vi "VIH Platform - LabVIEW - Read Show_Optional_Terminals status in Context Help.vi"(8 "error in":errorcluster) -> (0 "error out":errorcluster, 3 "simpleDiagramHelp (Hide Optional Terminals)":bool)   [LabVIEW 2014]
doc: "::: VI Helpeks :::\nCopyright (c) 2000-2026 Konstantin Shifershteyn. All rights reserved."
panel:
  # "VI Helpeks\nCopyright (c) 2012-2026 Konstantin Shifershteyn"
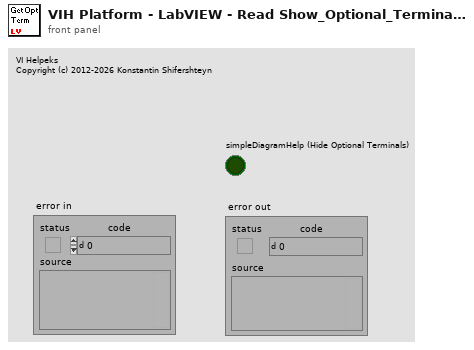
[diagram p1: front panel]
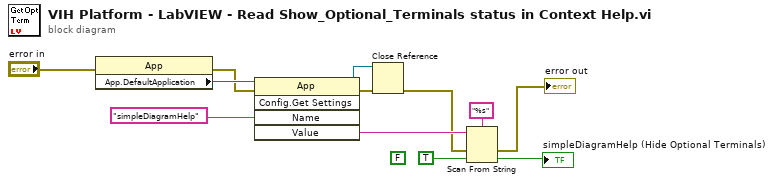
[diagram p0: block diagram]
diagram:
  (unwired) FALSE
  n1 = property class="App"(error in="error in") -> (error out=w10:errorcluster, "App.DefaultApplication"=w12:refnum<vi>)  [unwired: 1 in, 1 out]
  n2 = invoke class="App" method="Config.Get Settings"(reference=w12, error in=w10, "Name"="simpleDiagramHelp") -> (reference out=w9:refnum<vi>, error out=w8:errorcluster, "Value"=w7:string)  [unwired: 2 in, 2 out]
  n3 = Close Reference(reference=w9, error in (no error)=w8) -> (error out=w6:errorcluster)
  n4 = Scan From String(format string="%s", input string=w7, error in=w6, default 1=TRUE) -> (error out=→"error out":errorcluster, output 1=→"simpleDiagramHelp (Hide Optional Terminals)":bool)  [unwired: 1 in, 2 out]
